vi "GetAncestor Wrapper Template.vi"(0 "hwnd":u64, 5 "gaFlags":u32=2, 11 "error in":errorcluster) -> (4 "ancestor":u64, 15 "error out":errorcluster)   [LabVIEW 2020]
doc: "Returns an ancestor of the window hwnd through user32.dll GetAncestor (stdcall, called in any thread). gaFlags 2 GA_ROOT (default) gives the top-level window hwnd is part of, e.g. the dialog a focused edit control belongs to; 1 GA_PARENT the parent, 3 GA_ROOTOWNER the root window of the owner chain. ancestor is 0 when hwnd is not a window. When error in carries an error the DLL is not called. Generated by scripts\\Build Win32 Wrappers.vi - do not edit by hand, rebuild it."
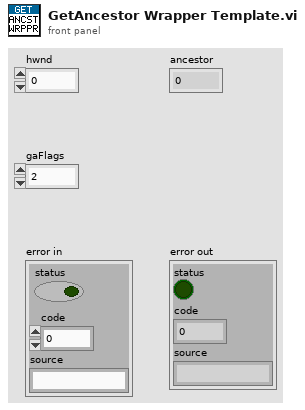
[diagram p1: front panel]
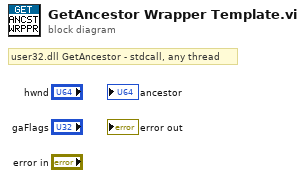
[diagram p0: block diagram]
diagram:
  # "user32.dll GetAncestor - stdcall, any thread"
